vi "Tree_AssertAllTags_Tests.vi"(11 "error in":errorcluster) -> (15 "error out":errorcluster)   [LabVIEW 2016, in "DronaTest.lvlib"]
uses:
  DronaTest.lvlib
  APIs/Stimulus/ControlValue/SetValueAuto.vi
  APIs/Assert/AssertControlValue/Controls/Tree/AssertAllTags.vi
  <vilib>/addons/_JKI Toolkits/Caraya/classes/Assert/Assert Error.vi
  <vilib>/addons/_JKI Toolkits/Caraya/classes/Assert/Assert Equal Value_Variant.vi
  <vilib>/addons/_JKI Toolkits/Caraya/classes/Test/Test.lvclass
  Drona.lvlib
  <vilib>/SLL Toolkit/SLL Debug/SLL Debug.lvlib
  <vilib>/addons/_JKI Toolkits/Caraya/classes/Assert/Assert.lvclass
  APIs/Stimulus/ControlValue/ControlValue.lvlib
  APIs/Assert/AssertControlValue/Controls/Tree/AssertTree.lvlib
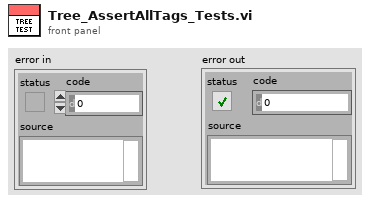
[diagram p1: front panel]
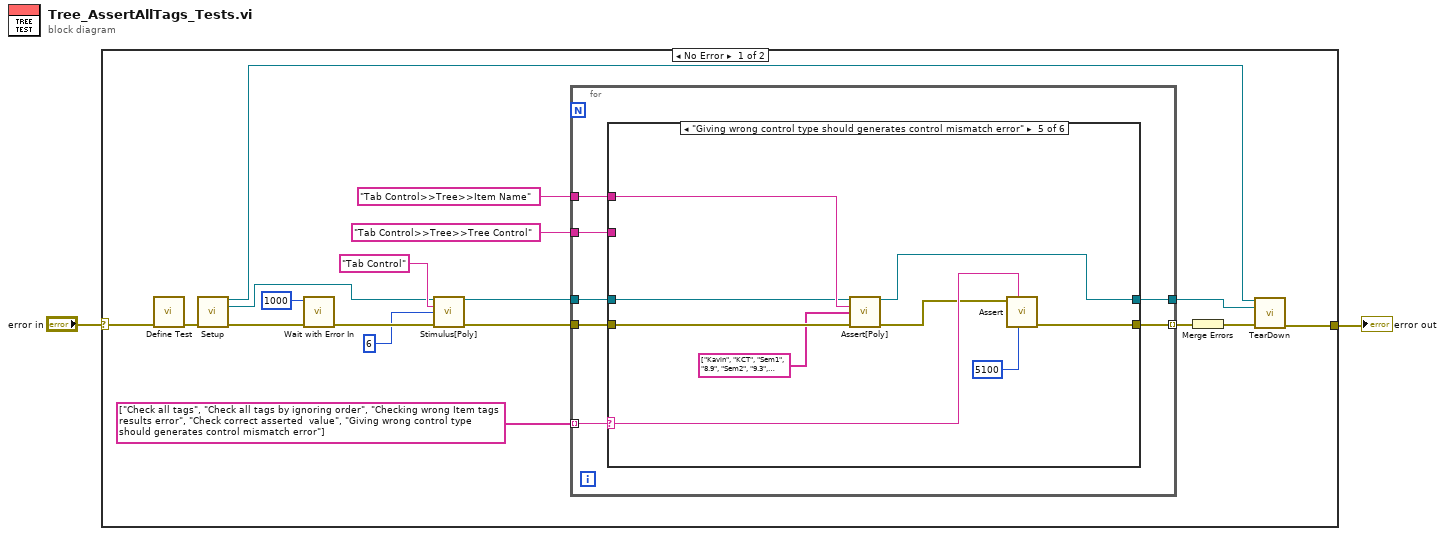
[diagram p0: block diagram]
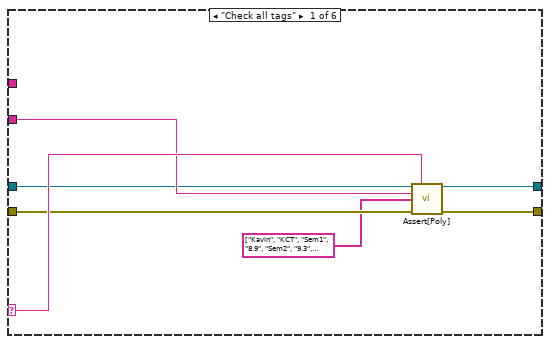
[diagram p2: hidden frame]
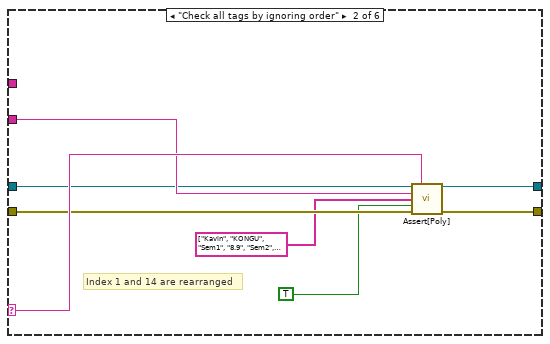
[diagram p3: hidden frame]
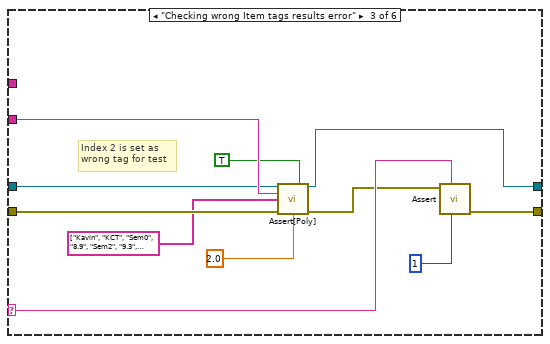
[diagram p4: hidden frame]
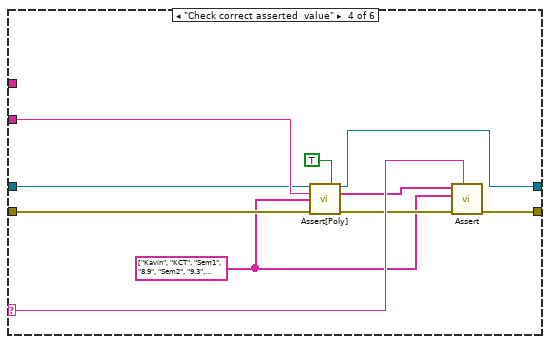
[diagram p5: hidden frame]
diagram:
  n1 = case shown="No Error" "error in" {
    selector: "error in" -> [w20 w75]
    tunnel: [w5 w75] -> w1
    frame No Error {
      n2 = call <vilib>:"Define Test.vi"("error in (no error)"=w20) -> ("error out"=w11:errorcluster)  [unwired: 9 in, 1 out]
      n3 = call "Setup.vi"("error in"=w11) -> ("Application Ref"=w7:refnum<vi>, "VI out"=w9:refnum<vi>, "error out"=w10:errorcluster)  [unwired: 12 in]
      n4 = call <vilib>:"Wait with Error In.vi"("error in (no error)"=w10, "milliseconds to wait"=u32 1000) -> ("error out"=w18:errorcluster)  [unwired: 9 in]
      n5 = call-poly "Stimulus[Poly].vi"("VI Reference In"=w9, "Control Path"="Tab Control", "Value (Signaling)"=6, "error in"=w18) -> ("VI Reference Out"=w14:refnum<vi>, "error out"=w17:errorcluster)  [unwired: 10 in]
      n6 = for {
        tunnel: w14 -> [w26]
        tunnel: "Tab Control>>Tree>>Tree Control" ("Control Path") -> [w25]
        tunnel: "Tab Control>>Tree>>Item Name" ("Control Path") -> [w24]
        tunnel: string[] ["Check all tags", "Check all tags by ignoring order", "Checking wrong Item tags results error", "Check correct asserted  value", "Giving wrong control type should generates control mismatch error"] -> [w22] mode=indexing
        tunnel: [w21] -> w6
        tunnel: w17 -> [w27]
        tunnel: [w23] -> w12 mode=indexing
        n7 = case shown="\"Giving wrong control type should generates control mismatch error\"" w22 {
          selector: w22 -> [w32 w40 w52 w62 w71 _]
          tunnel: w27 -> [w30 w38 w45 w58 w66 w74]
          tunnel: w26 -> [w29 w37 w44 w57 w65 w73]
          tunnel: w25 -> [w31 w39 w50 w61 _ _]
          tunnel: w24 -> [_ _ _ _ w68 _]
          tunnel: [w34 w42 w53 w63 w72 w74] -> w23
          tunnel: [w33 w41 w49 w60 w67 w73] -> w21
          frame "Check all tags" {
            n8 = call-poly "Assert[Poly].vi"("VI Reference In"=w29, "Test Label"=w32, "Control Path"=w31, "Item Tags"=string[] ["Kavin", "KCT", "Sem1", "8.9", "Sem2", "9.3", "Sem3", "9.3_1", "Sem4", "9.5", "Sem5", "9.2", "Sem6", "9.1", "KONGU", "Sem1_1", "8.8", "Sem2_1", "9.5_1", "Sem3_1", "9.6", "Sem4_1", "9.6_1", "Sem5_1", "9.4", "Sem6_1", "9.7"] ("All Tags"), "Error In"=w30) -> ("VI Reference Out"=w33:refnum<vi>, "Error Out"=w34:errorcluster)  [unwired: 8 in, 1 out]
          }
          frame "Check all tags by ignoring order" {
            # "Index 1 and 14 are rearranged"
            n9 = call-poly "Assert[Poly].vi"("VI Reference In"=w37, "Test Label"=w40, "Control Path"=w39, "Item Tags"=string[] ["Kavin", "KONGU", "Sem1", "8.9", "Sem2", "9.3", "Sem3", "9.3_1", "Sem4", "9.5", "Sem5", "9.2", "Sem6", "9.1", "KCT", "Sem1_1", "8.8", "Sem2_1", "9.5_1", "Sem3_1", "9.6", "Sem4_1", "9.6_1", "Sem5_1", "9.4", "Sem6_1", "9.7"] ("All Tags"), "Ignore Order? (F)"=TRUE, "Error In"=w38) -> ("VI Reference Out"=w41:refnum<vi>, "Error Out"=w42:errorcluster)  [unwired: 7 in, 1 out]
          }
          frame "Checking wrong Item tags results error" {
            # "Index 2 is set as \nwrong tag for test"
            n10 = call-poly "Assert[Poly].vi"("VI Reference In"=w44, "Assert Only? (F)"=TRUE, "Control Path"=w50, "Item Tags"=string[] ["Kavin", "KCT", "Sem0", "8.9", "Sem2", "9.3", "Sem3", "9.3_1", "Sem4", "9.5", "Sem5", "9.2", "Sem6", "9.1", "KONGU", "Sem1_1", "8.8", "Sem2_1", "9.5_1", "Sem3_1", "9.6", "Sem4_1", "9.6_1", "Sem5_1", "9.4", "Sem6_1", "9.7"] ("All Tags"), "Error In"=w45, "Timeout(5 sec)"=2.0) -> ("VI Reference Out"=w49:refnum<vi>, "Error Out"=w48:errorcluster)  [unwired: 7 in, 1 out]
            n11 = call-poly <vilib>:"Assert.vi"("error code (1)"=1, "Label"=w52, "Error?"=w48) -> ("error out"=w53:errorcluster)  [unwired: 7 in, 1 out]
          }
          frame "Check correct asserted  value" {
            w54 = string[] ["Kavin", "KCT", "Sem1", "8.9", "Sem2", "9.3", "Sem3", "9.3_1", "Sem4", "9.5", "Sem5", "9.2", "Sem6", "9.1", "KONGU", "Sem1_1", "8.8", "Sem2_1", "9.5_1", "Sem3_1", "9.6", "Sem4_1", "9.6_1", "Sem5_1", "9.4", "Sem6_1", "9.7"] ("All Tags")
            n12 = call-poly "Assert[Poly].vi"("VI Reference In"=w57, "Assert Only? (F)"=TRUE, "Control Path"=w61, "Item Tags"=w54, "Error In"=w58) -> ("VI Reference Out"=w60:refnum<vi>, "Asserted Value"=w55:string[], "Error Out"=w56:errorcluster)  [unwired: 8 in]
            n13 = call-poly <vilib>:"Assert.vi"("Label"=w62, "error in (no error)"=w56, "Y"=w54, "X"=w55) -> ("error out"=w63:errorcluster)  [unwired: 6 in, 1 out]
          }
          frame "Giving wrong control type should generates control mismatch error" {
            n14 = call-poly "Assert[Poly].vi"("VI Reference In"=w65, "Control Path"=w68, "Item Tags"=string[] ["Kavin", "KCT", "Sem1", "8.9", "Sem2", "9.3", "Sem3", "9.3_1", "Sem4", "9.5", "Sem5", "9.2", "Sem6", "9.1", "KONGU", "Sem1_1", "8.8", "Sem2_1", "9.5_1", "Sem3_1", "9.6", "Sem4_1", "9.6_1", "Sem5_1", "9.4", "Sem6_1", "9.7"] ("All Tags"), "Error In"=w66) -> ("VI Reference Out"=w67:refnum<vi>, "Error Out"=w69:errorcluster)  [unwired: 9 in, 1 out]
            n15 = call-poly <vilib>:"Assert.vi"("error code (1)"=5100, "Label"=w71, "Error?"=w69) -> ("error out"=w72:errorcluster)  [unwired: 7 in, 1 out]
          }
          frame Default {
          }
        }
      }
      n16 = Merge Errors(w12) -> (w8:errorcluster)
      n17 = call "TearDown.vi"("Application Ref"=w7, "VI in"=w6, "error in (no error)"=w8) -> ("error out"=w5:errorcluster)  [unwired: 12 in]
    }
    frame Error {
    }
  }
  "error out" <- w1
